vi "Set Mast Moving Speed.vi"(8 "error in (no error)":errorcluster, 11 "CO3000 in":refnum<class "CO3000.lvclass">) -> (0 "error out":errorcluster, 3 "CO3000 out":refnum<class "CO3000.lvclass">)   [LabVIEW 2023, in "Turn Table and Mast.lvlib" / "CO3000.lvclass"]
uses:
  CO3000.lvclass
  CO3000.lvclass/CO3000.ctl
panel:
  out "VISA Refnum out":refnum<visa-resource-name>
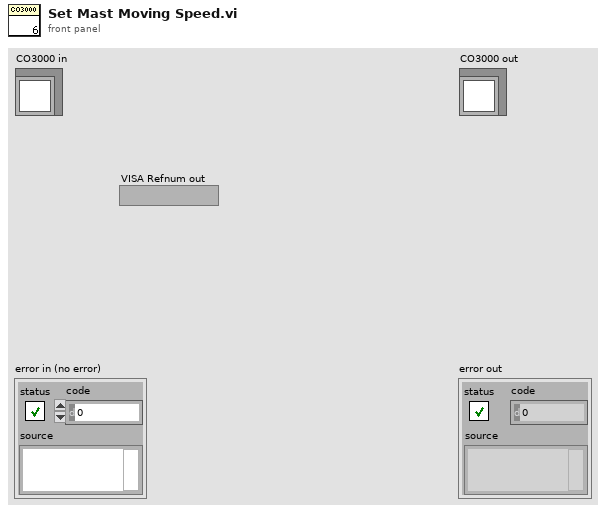
[diagram p1: front panel]
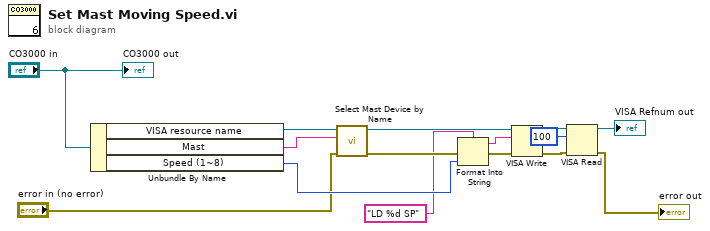
[diagram p0: block diagram]
diagram:
  n1 = Unbundle By Name("CO3000 in") -> ("VISA resource name"=w12:refnum<visa-resource-name>, "Mast"=w11:string, "Speed (1~8)"=w13:i32)
  n2 = call "Select Mast Device by Name.vi"("error in (no error)"="error in (no error)", "Mast Device"=w11, "VISA Refnum in"=w12) -> ("error out"=w8:errorcluster, "VISA Refnum out"=w10:refnum<visa-resource-name>)  [unwired: 7 in]
  n3 = Format Into String(format string="LD %d SP" ("버퍼 쓰기"), error in=w8, w13) -> (resulting string=w14:string, error out=w15:errorcluster)  [unwired: 1 in]
  n4 = VISA Write(VISA resource name=w10, write buffer=w14, error in (no error)=w15) -> (VISA resource name out=w6:refnum<visa-resource-name>, error out=w5:errorcluster)  [unwired: 1 out]
  n5 = VISA Read(VISA resource name=w6, byte count=u32 100, error in (no error)=w5) -> (VISA resource name out=→"VISA Refnum out":refnum<visa-resource-name>, error out=→"error out":errorcluster)  [unwired: 2 out]
  "CO3000 out" <- "CO3000 in"
